vi "Sim_IO_Adapter.vi"(8 "error in (no error)":errorcluster={"status"=FALSE, "code"=0, "source"="\"\""}, 10 "current_ms":i64, 11 "command_val":dbl=10.0) -> (0 "error out":errorcluster={"status"=FALSE, "code"=0, "source"="\"\""}, 1 "is_applied":bool, 2 "ack_time_ms":i64, 3 "feedback_val":dbl)   [LabVIEW 2026]
doc: "INTENT: Simulated I/O adapter validating synthetic commands and generating simulated feedback timestamps."
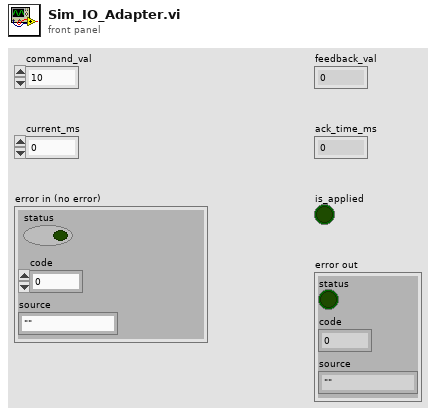
[diagram p1: front panel]
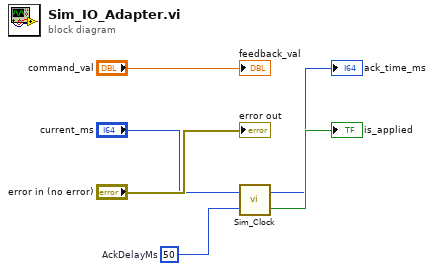
[diagram p0: block diagram]
diagram:
  w4 = i64 50  # AckDelayMs
  n1 = call "Sim_Clock.vi"("advance_ms"=w4, "current_ms"="current_ms") -> ("valid"=→"is_applied":bool, "next_ms"=→"ack_time_ms":i64)
  "feedback_val" <- "command_val"
  "error out" <- "error in (no error)"
